vi "query HO UL_DL Channel BandWidth.vi"(8 "error in (no error)":errorcluster caption="에러 입력(에러 없음)", 9 "Direction":T1, 10 "Bandwidth Setting Param":T2, 11 "NR 입력":refnum<class "NR.lvclass">) -> (0 "error out":errorcluster caption="에러 출력", 2 "BW (MHz)":u32, 3 "NR 출력":refnum<class "NR.lvclass">)   [LabVIEW 2023, in "ANRITSU Call Box.lvlib" / "NR.lvclass"]
uses:
  NR.lvclass
  NR.lvclass/NR.ctl
  Type Definition/Uplink Downlink Enum.ctl
  ANRITSU Call Box.lvlib
  Type Definition/NR Channel Bandwidth Param.ctl
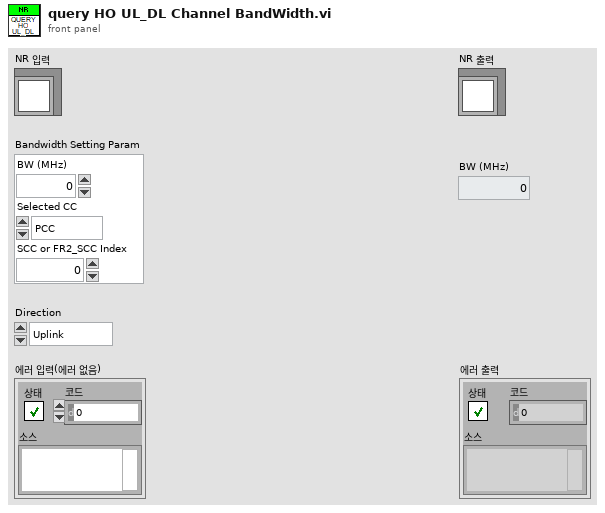
[diagram p1: front panel]
types:
  T1 = typedef "ANRITSU Call Box.lvlib/Uplink Downlink Enum.ctl" = enum16{"Uplink", "Downlink"}
  T2 = typedef "ANRITSU Call Box.lvlib/NR Channel Bandwidth Param.ctl" = cluster{"BW (MHz)":u32, "Selected CC":enum16{"PCC", "SCC", "FR2_PCC", "FR2_SCC"}, "SCC or FR2_SCC Index":u32}
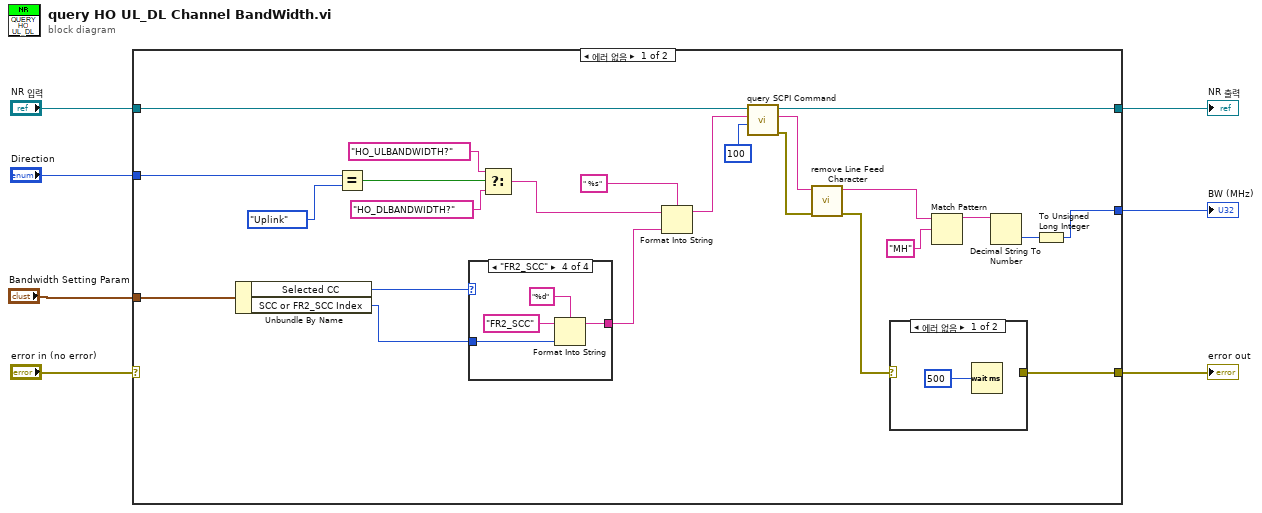
[diagram p0: block diagram]
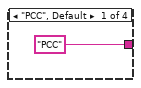
[diagram p3: hidden frame]
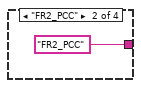
[diagram p4: hidden frame]
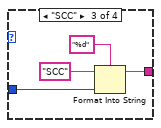
[diagram p5: hidden frame]
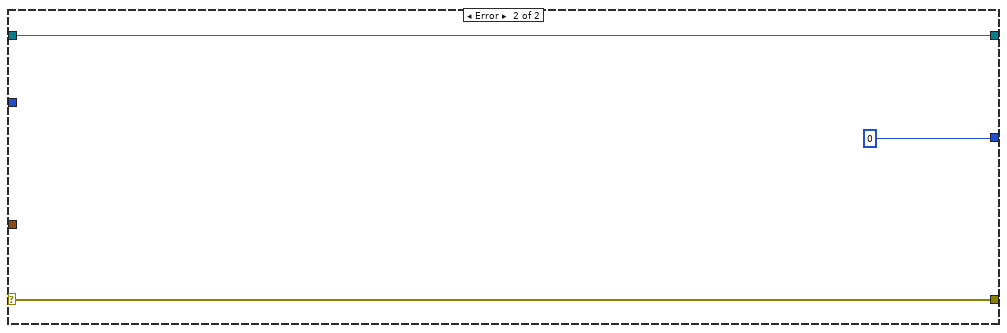
[diagram p6: hidden frame]
diagram:
  n1 = case shown="에러 없음" "error in (no error)" {
    selector: "error in (no error)" -> [_ w46]
    tunnel: [w11 w46] -> w6
    tunnel: [w13 w45] -> w4
    tunnel: "NR 입력" -> [w14 w45]
    tunnel: [w12 u32 0] -> w3
    tunnel: "Bandwidth Setting Param" -> [w10 _]
    tunnel: "Direction" -> [w8 _]
    frame No Error {
      n2 = Unbundle By Name(w10) -> ("Selected CC"=w9:enum16{"PCC", "SCC", "FR2_PCC", "FR2_SCC"}, "SCC or FR2_SCC Index"=w27:u32)
      n3 = Equal?(x=w8, y=Uplink_Downlink_Enum."Uplink") -> (x = y?=w28:bool)
      n4 = case shown="\"FR2_SCC\"" w9 {
        tunnel: ["PCC" "FR2_PCC" w37 w41] -> w25
        tunnel: w27 -> [_ _ w36 w40]
        frame "PCC", Default {
        }
        frame "FR2_PCC" {
        }
        frame "SCC" {
          n5 = Format Into String(format string="%d", initial string="SCC", w36) -> (resulting string=w37:string)  [unwired: 1 in, 1 out]
        }
        frame "FR2_SCC" {
          n6 = Format Into String(format string="%d", initial string="FR2_SCC", w40) -> (resulting string=w41:string)  [unwired: 1 in, 1 out]
        }
      }
      n7 = Select(t="HO_ULBANDWIDTH?" ("format string"), s=w28, f="HO_DLBANDWIDTH?" ("format string")) -> (s? t:f=w26:string)
      n8 = Format Into String(format string=" %s", initial string=w26, w25) -> (resulting string=w18:string)  [unwired: 1 in, 1 out]
      n9 = call "query SCPI Command.vi"("Read Buffer Length"=u32 100, "SCPI Command"=w18, "NR in"=w14) -> ("error out"=w15:errorcluster, "Read Buffer String"=w16:string, "NR out"=w13:refnum<class "NR.lvclass">)  [unwired: 6 in]
      n10 = call "remove Line Feed Character.vi"("error in"=w15, "Query String"=w16) -> ("error out"=w19:errorcluster, "Line Feed Removed String"=w21:string)  [unwired: 8 in]
      n11 = case shown="에러 없음" w19 {
        selector: w19 -> [_ w33]
        tunnel: [_ w33] -> w11
        frame No Error {
          n12 = Wait (ms)(milliseconds to wait=u32 500) -> ()  [unwired: 1 out]
        }
        frame Error {
        }
      }
      n13 = Match Pattern(string=w21, regular expression="MH") -> (before substring=w23:string)  [unwired: 1 in, 3 out]
      n14 = Decimal String To Number(string=w23) -> (number=w22:i32)  [unwired: 2 in, 1 out]
      n15 = To Unsigned Long Integer(number=w22) -> (unsigned 32bit integer=w12:u32)
    }
    frame Error {
    }
  }
  "error out" <- w6
  "NR 출력" <- w4
  "BW (MHz)" <- w3
